vi "GetTemplatePath.vi"(0 "reference in":refnum<class "ClassWriterNative.lvclass">, 1 "ClassTemplateSubDirectory":string, 5 "error in (no error)":errorcluster) -> (14 "reference out":refnum<class "ClassWriterNative.lvclass">, 15 "FolderPathOut":path, 17 "MethodTemplatePathOut":path, 18 "TemplateSettings":T1, 19 "error out":errorcluster)   [LabVIEW 2020, in "ClassWriterNative.lvclass"]
uses:
  <resource>/Framework/Providers/Open_GDS/ClassProviders/Provider_LvNativeClass/ClassWriterNative_class/ClassWriterNative.lvclass
  <resource>/Framework/Providers/Open_GDS/ClassProviders/Provider_BaseClassInterface/ClassWriter_class/TemplateSettings.ctl
  <resource>/Framework/Providers/Open_GDS/ClassProviders/Provider_LvNativeClass/ClassWriterNative_class/ClassWriterNative.lvclass/ClassWriterNative.ctl
  <resource>/Framework/Providers/Open_GDS/ClassProviders/Provider_BaseClassInterface/ClassWriter_class/ClassWriter.lvclass
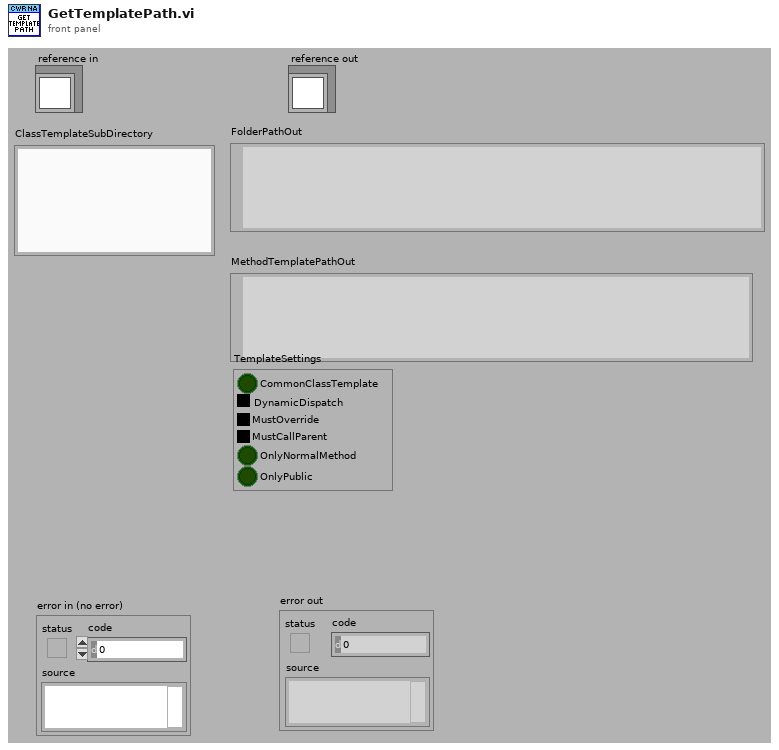
[diagram p1: front panel]
types:
  T1 = typedef "ClassWriter.lvclass/TemplateSettings.ctl" = cluster{"CommonClassTemplate":bool, "DynamicDispatch":enum8{"False", "True", "Mixed"}, "MustOverride":enum8{"False", "True", "Mixed"}, "MustCallParent":enum8{"False", "True", "Mixed"}, "OnlyNormalMethod":bool, "OnlyPublic":bool}
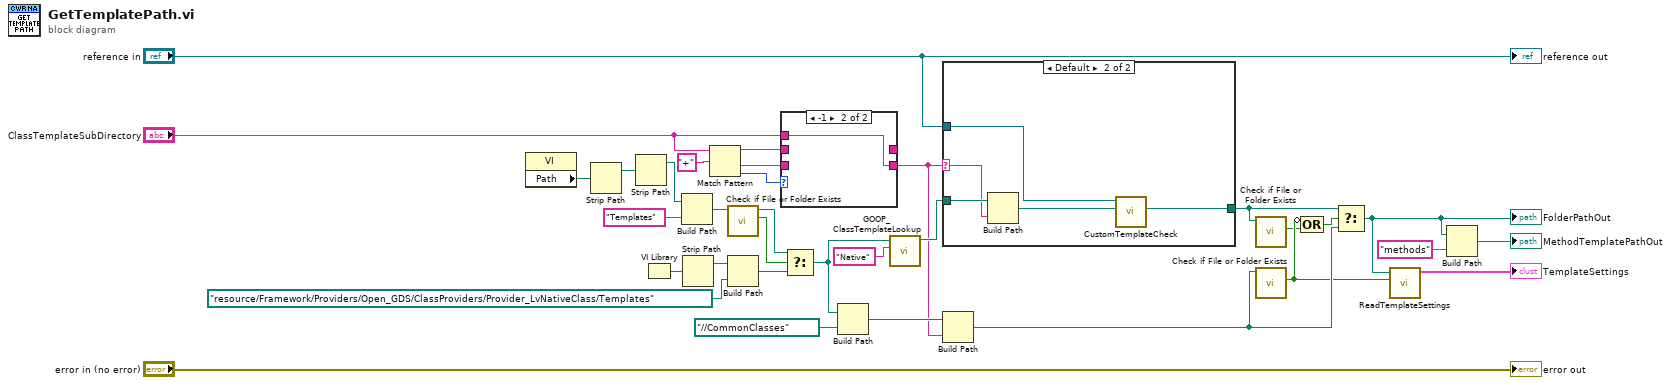
[diagram p0: block diagram]
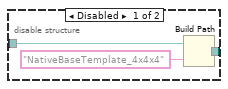
[diagram p4: hidden frame]
diagram:
  n1 = property class="VI"() -> ("Path"=w31:path)  [unwired: 2 in, 2 out]
  n2 = Strip Path(path=w31) -> (stripped path=w29:path)  [unwired: 1 out]
  n3 = Strip Path(path=w29) -> (stripped path=w33:path)  [unwired: 1 out]
  n4 = VI Library() -> (path=w25:path)
  n5 = Build Path(base path=w33, name or relative path="Templates") -> (appended path=w26:path)
  n6 = Strip Path(path=w25) -> (stripped path=w21:path)  [unwired: 1 out]
  n7 = Match Pattern(string="ClassTemplateSubDirectory", regular expression="+") -> (before substring=w17:string, after substring=w20:string, offset past match=w19:i32)  [unwired: 1 in, 1 out]
  n8 = call <vilib>:"Check if File or Folder Exists.vi"("path"=w26) -> ("file or folder exists?"=w28:bool, "dup path"=w27:path)  [unwired: 8 in, 1 out]
  n9 = Build Path(base path=w21, name or relative path=path "resource/Framework/Providers/Open_GDS/ClassProviders/Provider_LvNativeClass/Templates") -> (appended path=w24:path)
  n10 = case shown="-1" w19 {
    tunnel: "ClassTemplateSubDirectory" -> [_ w36]
    tunnel: [w35 w36] -> w10
    tunnel: w20 -> [w35 _]
    tunnel: [w34 _] -> _
    tunnel: w17 -> [w34 _]
    frame 0, Default {
    }
    frame -1 {
    }
  }
  n11 = Select(t=w27, s=w28, f=w24) -> (s? t:f=w12:path)
  n12 = Build Path(base path=w12, name or relative path=path "../../CommonClasses") -> (appended path=w11:path)
  n13 = call <resource>:"GOOP_ClassTemplateLookup.vi"("ClassType"="Native", "ClassTemplateFolderIn"=w12) -> ("ClassTemplateFolderOut"=w15:path)  [unwired: 9 in]
  n14 = case shown="Default" w10 {
    selector: w10 -> [_ w46]
    tunnel: w15 -> [w38 w47]
    tunnel: [w37 w43] -> w13
    tunnel: "reference in" -> [_ w45]
    frame "" {
      # "Not sure why we needed to add a default class\nif Template is empty.\nWe need this way to get the Root folder of all \nBuild in Templates"
      n15 = disable-structure shown="Enabled" {
        disable-tunnel: w38 -> [w41 w42]
        disable-tunnel: [w40 w42] -> w37
        frame Disabled {
          n16 = Build Path(base path=w41, name or relative path="NativeBaseTemplate_4x4x4") -> (appended path=w40:path)
        }
        frame Enabled {
        }
      }
    }
    frame Default {
      n17 = Build Path(base path=w47, name or relative path=w46) -> (appended path=w44:path)
      n18 = call <resource>:"CustomTemplateCheck.vi"("ClassTemplate"=w44, "ClassWriterNative in"=w45) -> ("ClassTemplate(Maybe Modified if not exists)"=w43:path)  [unwired: 9 in]
    }
  }
  n19 = Build Path(base path=w11, name or relative path=w10) -> (appended path=w5:path)
  n20 = call <vilib>:"Check if File or Folder Exists.vi"("path"=w13) -> ("file or folder exists?"=w3:bool)  [unwired: 8 in, 2 out]
  n21 = call <vilib>:"Check if File or Folder Exists.vi"("path"=w5) -> ("file or folder exists?"=w4:bool)  [unwired: 8 in, 2 out]
  n22 = Compound Arithmetic op=OR(invert w4, w3) -> (w2:bool)
  n23 = Select(t=w13, s=w2, f=w5) -> (s? t:f=w6:path)
  "FolderPathOut" <- w6
  n24 = call <resource>:"ReadTemplateSettings.vi"("CommonClassTemplate"=w4, "TemplateFolder"=w6) -> ("TemplateSettings"=→"TemplateSettings":T1)  [unwired: 9 in]
  n25 = Build Path(base path=w6, name or relative path="methods") -> (appended path=→"MethodTemplatePathOut":path)
  "error out" <- "error in (no error)"
  "reference out" <- "reference in"
